vi "Delete Data Folder.vi"(5 "Files Generated by Build":path[](array[path]), 6 "Top Level/Always Included VIs":path[](array[path]), 7 "Destination Path":path, 8 "error in (no error)":errorcluster, 9 "Target Name":string, 10 "Build Specification Name":string, 11 "Project Path":path) -> (0 "error out":errorcluster)   [LabVIEW 2020, in "Build VIs.lvlib"]
uses:
  Build VIs.lvlib
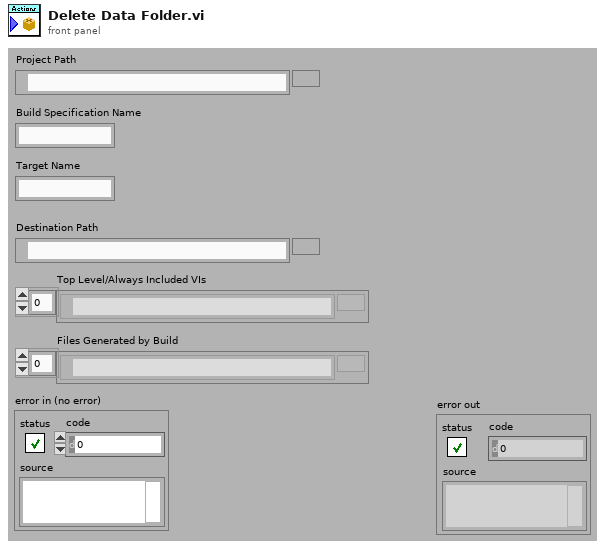
[diagram p1: front panel]
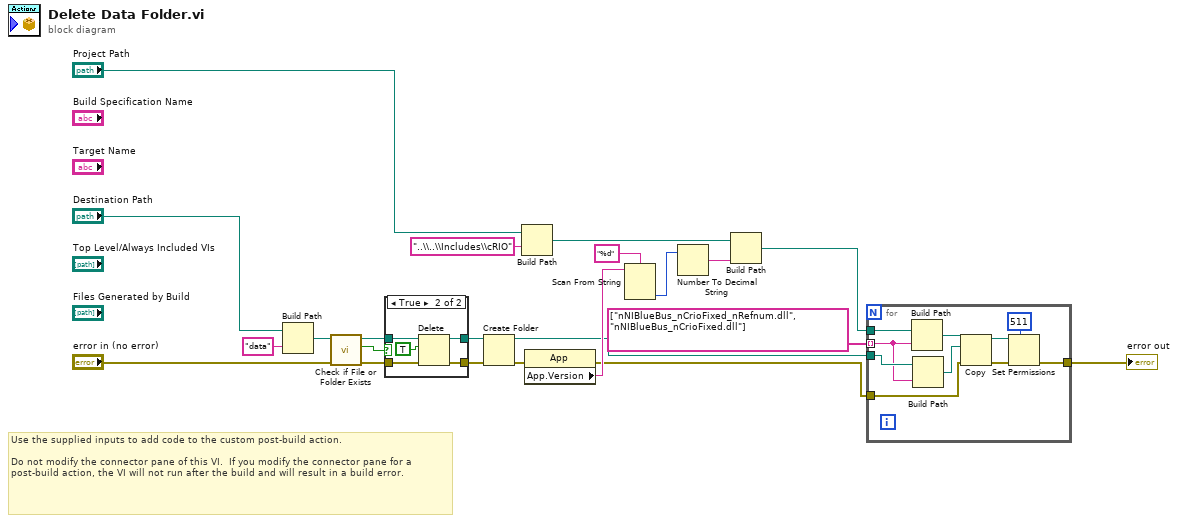
[diagram p0: block diagram]
diagram:
  # "Use the supplied inputs to add code to the custom post-build action.\n\nDo not modify the connector pane of this VI.  If you modify the connector pane for a post-build action, the VI will not run after the build and will result in a build error."
  n1 = Build Path(base path="Destination Path", name or relative path="data") -> (appended path=w20:path)
  n2 = call <vilib>:"Check if File or Folder Exists.vi"("error in (no error)"="error in (no error)", "path"=w20) -> ("error out"=w18:errorcluster, "file or folder exists?"=w19:bool, "dup path"=w13:path)  [unwired: 7 in]
  n3 = case shown="True" w19 {
    tunnel: w13 -> [w23 w29]
    tunnel: w18 -> [w24 w27]
    tunnel: [w24 w26] -> w15
    tunnel: [w23 w25] -> w12
    frame False {
    }
    frame True {
      n4 = Delete(path (use dialog)=w29, entire hierarchy (F)=TRUE, error in=w27) -> (deleted path=w25:path, error out=w26:errorcluster)  [unwired: 2 in, 1 out]
    }
  }
  n5 = Create Folder(path (use dialog)=w12, error in=w15) -> (created path=w1:path, error out=w14:errorcluster)  [unwired: 1 in, 1 out]
  n6 = Build Path(base path="Project Path", name or relative path="..\\..\\Includes\\cRIO") -> (appended path=w9:path)
  n7 = property class="App"(error in=w14) -> (error out=w4:errorcluster, "App.Version"=w17:string)  [unwired: 1 in, 1 out]
  n8 = Scan From String(format string="%d", input string=w17) -> (output 1=w8:i32)  [unwired: 3 in, 3 out]
  n9 = Number To Decimal String(number=w8) -> (decimal integer string=w7:string)  [unwired: 1 in]
  n10 = Build Path(base path=w9, name or relative path=w7) -> (appended path=w5:path)
  n11 = for {
    tunnel: string[] ["nNIBlueBus_nCrioFixed_nRefnum.dll", "nNIBlueBus_nCrioFixed.dll"] -> [w30] mode=indexing
    tunnel: w5 -> [w39]
    tunnel: w4 -> [w37]
    tunnel: [w33] -> w2
    tunnel: w1 -> [w31]
    n12 = Build Path(base path=w39, name or relative path=w30) -> (appended path=w38:path)
    n13 = Build Path(base path=w31, name or relative path=w30) -> (appended path=w32:path)
    n14 = Copy(8:w37, 10:w32, 11:w38) -> (0:w34:errorcluster, 3:w35:path)  [unwired: 2 in, 1 out]
    n15 = Set Permissions(7:i16 511 ("permissions"), 8:w34, 11:w35) -> (0:w33:errorcluster)  [unwired: 2 in, 1 out]
  }
  "error out" <- w2
